vi "Update Lua Palettes.vi"() -> ()   [LabVIEW 2020, in "Lua DevUtil.lvlib"]
uses:
  Lua DevUtil.lvlib
  <vilib>/Utility/miscctls.llb/LVMapReplaceAction.ctl
  <vilib>/Palette API/Palette Menu/Public Type Define/Palette Data.ctl
  <vilib>/Palette API/Palette Menu/Public Type Define/View Format.ctl
  <vilib>/Palette API/Palette Menu/Public Type Define/Items.ctl
  <vilib>/Palette API/Palette Menu/Public Type Define/Item.ctl
  <vilib>/Palette API/Palette Menu/Public Type Define/Help Info.ctl
  <vilib>/Palette API/Palette Menu/Public Type Define/Synchronize Info.ctl
  <vilib>/Palette API/Palette Menu/Public Type Define/Palette type.ctl
  85e9b90b-9151-4f09-9030-f452b0e3cf19.vi
  <vilib>/Comparison/Less/Less Functor/Less Functor.lvclass
  <vilib>/Palette API/Palette Menu/Palette Menu.lvlib
panel:
  out "errors":T1(array[cluster])
  out "Lua menus":T2(c390)
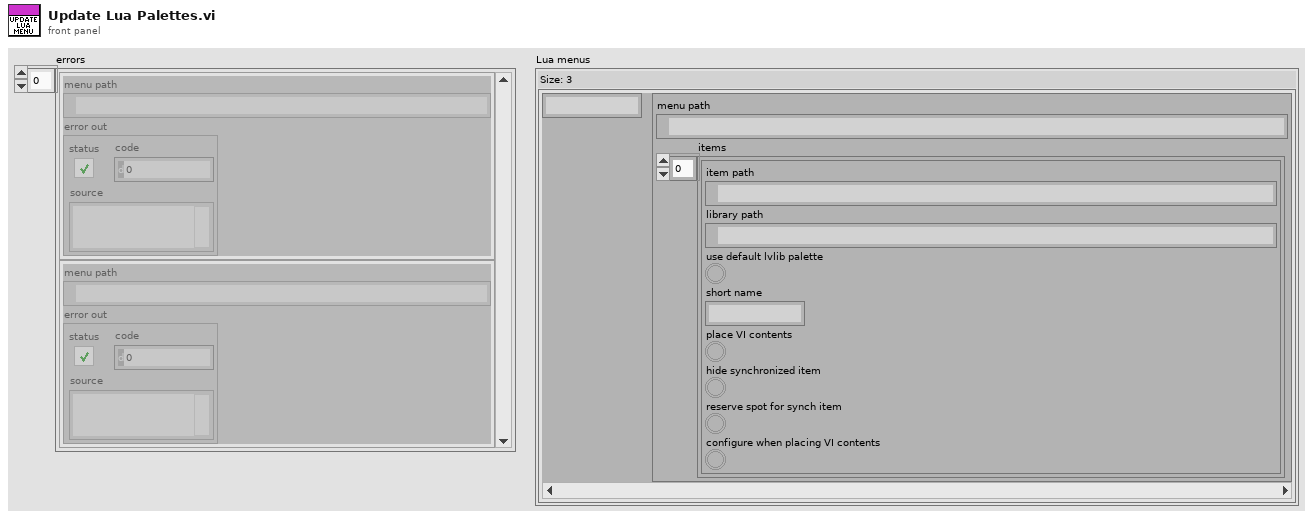
[diagram p1: front panel]
types:
  T1 = cluster{"menu path":path, "error out":errorcluster}[]
  T2 = map{string, cluster{"menu path":path, "items":cluster{"item path":path, "library path":path, "use default lvlib palette":bool, "short name":string, "place VI contents":bool, "hide synchronized item":bool, "reserve spot for synch item":bool, "configure when placing VI contents":bool}[]}}
  T3 = cluster{"item path":path, "library path":path, "use default lvlib palette":bool, "short name":string, "place VI contents":bool, "hide synchronized item":bool, "reserve spot for synch item":bool, "configure when placing VI contents":bool}
  T4 = typedef "LVMapReplaceAction.ctl" = enum32{"Modify Entry only if found", "Add or Modify Entry", "Delete Entry"}
  T5 = cluster{"menu path":path, "items":cluster{"item path":path, "library path":path, "use default lvlib palette":bool, "short name":string, "place VI contents":bool, "hide synchronized item":bool, "reserve spot for synch item":bool, "configure when placing VI contents":bool}[]}
  T6 = cluster{"item path":path, "library path":path, "use default lvlib palette":bool, "short name":string, "place VI contents":bool, "hide synchronized item":bool, "reserve spot for synch item":bool, "configure when placing VI contents":bool}[]
  T7 = typedef "Palette Menu.lvlib/View Format.ctl" = u16
  T8 = typedef "Palette Menu.lvlib/Palette Data.ctl" = cluster{"display name":string, "view format":T7, "palette width":i16, "items":T9, "256 color icon":picture, "B&W color icon":picture, "help information":T11, "palette description":string, "synchronize information":T12}
  T9 = typedef "Palette Menu.lvlib/Items.ctl" = T10[]
  T10 = typedef "Palette Menu.lvlib/Item.ctl" = cluster{"item path":path, "library path":path, "use default lvlib palette":bool, "short name":string, "place VI contents":bool, "hide synchronized item":bool, "reserve spot for synch item":bool, "configure when placing VI contents":bool}
  T11 = typedef "Palette Menu.lvlib/Help Info.ctl" = cluster{"help tag":string, "help file path ":path}
  T12 = typedef "Palette Menu.lvlib/Synchronize Info.ctl" = cluster{"synchronize with directory":bool, "synchronize directory path":path}
  T13 = typedef "Palette Menu.lvlib/Palette type.ctl" = i32
  T14 = cluster{"menu path":path, "error out":errorcluster}
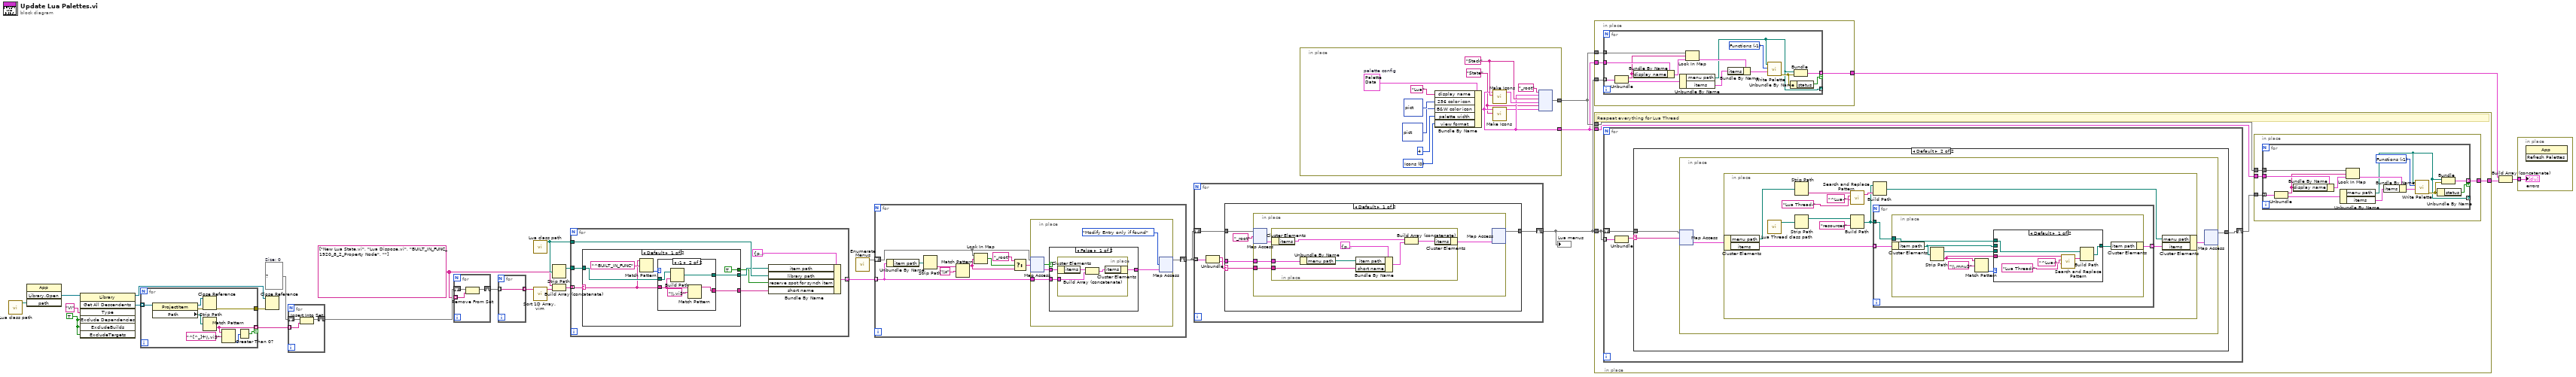
[diagram p0: block diagram]
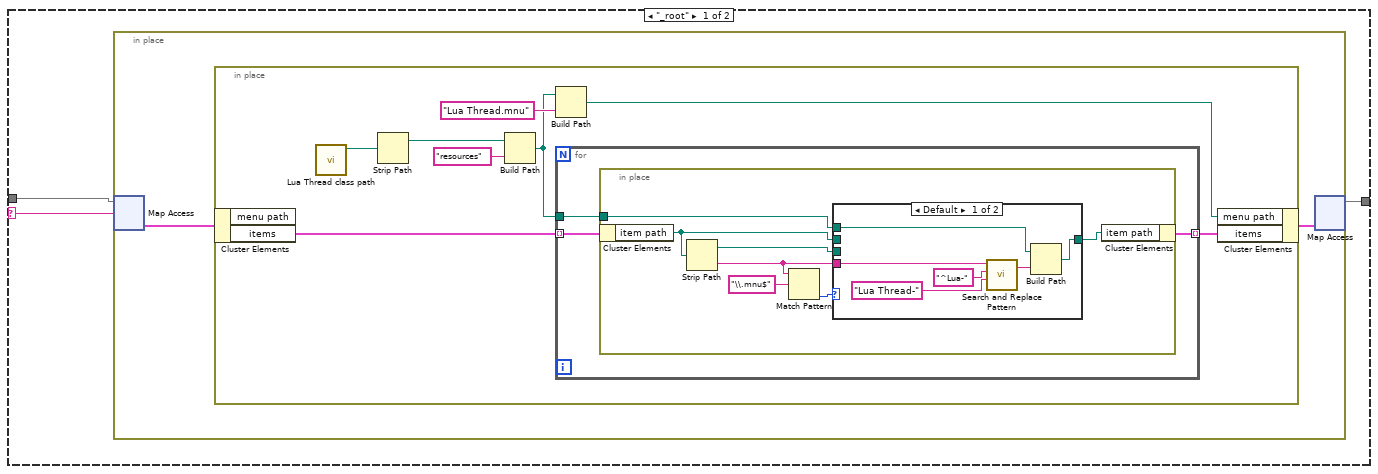
[diagram p2: hidden frame]
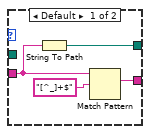
[diagram p7: hidden frame]
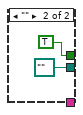
[diagram p8: hidden frame]
diagram:
  w17 = set{string} {}  # Size: 0
  w22 = TRUE ("ExcludeDependencies")
  w7 = string[] ["New Lua State.vi", "Lua Dispose.vi", "BUILT_IN_FUNC_1920_8_2_Property Node", ""]
  n1 = call "Lua class path.vi"() -> ("palette file path"=w25:path)  [unwired: 11 in]
  n2 = invoke class="App" method="Library.Open"("path"=w25) -> ("Open Library"=w24:refnum<vi>)  [unwired: 3 in, 3 out]
  n3 = invoke class="Library" method="Get All Descendents"(reference=w24, "Type"="VI", "Exclude Dependencies"=w22, "ExcludeBuilds"=w22, "ExcludeTargets"=w22) -> (reference out=w20:refnum<vi>, "All Descendents"=w21:refnum<vi>[])  [unwired: 2 in, 5 out]
  n4 = for {
    tunnel: w21 -> [w35] mode=indexing
    tunnel: [w27] -> w18 mode=indexing if=w29
    tunnel: [w32] -> w19
    n5 = property class="ProjectItem"(reference=w35) -> (reference out=w33:refnum<vi>, error out=w34:errorcluster, "Path"=w28:path)  [unwired: 1 in]
    n6 = Close Reference(reference=w33, error in (no error)=w34) -> (error out=w32:errorcluster)
    n7 = Strip Path(path=w28) -> (name=w27:string)  [unwired: 1 out]
    n8 = Match Pattern(string=w27, regular expression="^[^_]+\\.vi$") -> (offset past match=w30:i32)  [unwired: 1 in, 3 out]
    n9 = Greater Than 0?(x=w30) -> (x > 0?=w29:bool)
  }
  n10 = Close Reference(reference=w20, error in (no error)=w19) -> ()  [unwired: 1 out]
  n11 = for {
    shift-right: [w38] -> w16
    shift-left: w17 -> [w36]
    tunnel: w18 -> [w37] mode=indexing
    n12 = Insert Into Set(10:w37, 11:w36) -> (3:w38:set{string})  [unwired: 1 out]
  }
  n13 = for {
    shift-right: [w40] -> w15
    shift-left: w16 -> [w41]
    tunnel: w7 -> [w39] mode=indexing
    n14 = Remove From Set(10:w39, 11:w41) -> (3:w40:set{string})  [unwired: 1 out]
  }
  n15 = for {
    tunnel: w15 -> [w42] mode=indexing
    tunnel: [w42] -> w14 mode=indexing
  }
  n16 = call "Lua class path.vi"() -> ("palette file path"=w26:path)  [unwired: 11 in]
  n17 = call "Sort 1D Array.vim"("unsorted array"=w14) -> ("sorted array"=w13:string[])  [unwired: 10 in]
  n18 = Strip Path(path=w26) -> (stripped path=w11:path)  [unwired: 1 out]
  n19 = Build Array (concatenate)(w7, w13) -> (w12:string[])
  n20 = for {
    tunnel: w12 -> [w48] mode=indexing
    tunnel: [w49] -> w9 mode=indexing
    tunnel: w26 -> [w47]
    tunnel: w11 -> [w46]
    n21 = case shown="Default" w48 {
      selector: w48 -> [w54 _]
      tunnel: w46 -> [w57 _]
      tunnel: [w53 path "" ("appended path")] -> w45
      tunnel: [w52 _] -> w44
      tunnel: [TRUE ("use default lvlib palette") TRUE ("use default lvlib palette")] -> w43
      frame Default {
        n22 = Match Pattern(string=w54, regular expression="^BUILT_IN_FUNC") -> (offset past match=w55:i32)  [unwired: 1 in, 3 out]
        n23 = case shown="-1" w55 {
          tunnel: w57 -> [_ w66]
          tunnel: w54 -> [w60 w64]
          tunnel: [w61 w65] -> w53
          tunnel: [w58 w62] -> w52
          frame Default {
            n24 = String To Path(string=w60) -> (path=w61:path)
            n25 = Match Pattern(string=w60, regular expression="[^_]+$") -> (match substring=w58:string)  [unwired: 1 in, 3 out]
          }
          frame -1 {
            n26 = Build Path(base path=w66, name or relative path=w64) -> (appended path=w65:path)
            n27 = Match Pattern(string=w64, regular expression="\\.vi$") -> (before substring=w62:string)  [unwired: 1 in, 3 out]
          }
        }
      }
      frame "" {
      }
    }
    n28 = Bundle By Name(cluster=T3 {"item path"=path "", "library path"=path "", "use default lvlib palette"=FALSE, "short name"="", "place VI contents"=FALSE, "hide synchronized item"=FALSE, "reserve spot for synch item"=TRUE, "configure when placing VI contents"=FALSE}, "item path"=w45, "library path"=w47, "reserve spot for synch item"=w43, "short name"=w44) -> (w49:T3)
  }
  n29 = call "Enumerate Menus.vi"() -> ("Lua menus"=w10:T2)  [unwired: 11 in]
  n30 = for {
    shift-right: [w75] -> w8
    shift-left: w10 -> [w73]
    tunnel: w9 -> [w74] mode=indexing
    n31 = Unbundle By Name(w74) -> ("item path"=w78:path)
    n32 = Strip Path(path=w78) -> (name=w77:string)  [unwired: 1 out]
    n33 = Match Pattern(string=w77, regular expression="\\s") -> (before substring=w71:string)  [unwired: 1 in, 3 out]
    n34 = Look In Map(map=w73, key=w71) -> (key not found?=w72:bool)  [unwired: 1 in, 1 out]
    n35 = Select(t="_root" ("regular expression"), s=w72, f=w71) -> (s? t:f=w69:string)
    n36 = in-place {
      in-place-border: w74 -> [w79]
      n37 = in-place-map #1(w73, w69) -> (w81:T5, w83:bool)  [unwired: 1 in]
      n38 = case shown="False" w83 {
        tunnel: [w84 w90] -> w82
        tunnel: w81 -> [w86 w90]
        tunnel: w79 -> [w85 _]
        frame False {
          n39 = in-place {
            in-place-border: w85 -> [w88]
            n40 = in-place-cluster #2(w86) -> ("items"=w89:T6)
            n41 = Build Array (concatenate)(w89, w88) -> (w87:T6)
            n42 = in-place-cluster #2("items"=w87) -> (w84:T5)
          }
        }
        frame True {
        }
      }
      n43 = in-place-map #1(w82, LVMapReplaceAction."Modify Entry only if found" ("action")) -> (w75:T2)  [unwired: 2 out]
    }
  }
  n44 = for {
    tunnel: w8 -> [w95] mode=indexing
    shift-right: [w92] -> w5
    shift-left: w8 -> [w93]
    n45 = Unbundle(w95) -> ("submatch 1"=w94:string, w91:T5)
    n46 = case shown="Default" w94 {
      selector: w94 -> [w97 _]
      tunnel: w93 -> [w100 w112]
      tunnel: [w98 w112] -> w92
      tunnel: w91 -> [w99 _]
      frame Default {
        n47 = in-place {
          in-place-border: w99 -> [w103]
          in-place-border: w97 -> [w101]
          n48 = in-place-map #3(w100, "_root") -> (w104:T5)  [unwired: 1 in, 1 out]
          n49 = in-place {
            in-place-border: w103 -> [w111]
            in-place-border: w101 -> [w106]
            n50 = in-place-cluster #4(w104) -> ("items"=w110:T6)
            n51 = Unbundle By Name(w111) -> ("menu path"=w107:path)
            n52 = Bundle By Name(cluster=T3 {"item path"=path "", "library path"=path "", "use default lvlib palette"=FALSE, "short name"="", "place VI contents"=FALSE, "hide synchronized item"=FALSE, "reserve spot for synch item"=FALSE, "configure when placing VI contents"=FALSE}, "item path"=w107, "short name"=w106) -> (w105:T3)
            n53 = Build Array (concatenate)(w110, w105) -> (w109:T6)
            n54 = in-place-cluster #4("items"=w109) -> (w102:T5)
          }
          n55 = in-place-map #3(w102) -> (w98:T2)  [unwired: 1 in, 2 out]
        }
      }
      frame "_root" {
      }
    }
  }
  "Lua menus" <- w5
  n56 = in-place {
    in-place-border: [w119] -> w2
    in-place-border: [w115] -> w1
    w114 = "State" ("key")
    w118 = T7 0 items=["Icons", "Text", "Icons and Text"] ("view format")
    w116 = "Stack" ("key")
    w125 = T8 {"display name"="Lua", "view format"=0, "palette width"=2, "items"=[], "256 color icon"=bytes[1182], "B&W color icon"=bytes[286], "help information"={"help tag"="", "help file path "=path ""}, "palette description"="", "synchronize information"={"synchronize with directory"=FALSE, "synchronize directory path"=path ""}}  # palette config
    n57 = Bundle By Name(cluster=w125, "display name"="Lua", "256 color icon"=picture bytes[1182], "B&W color icon"=picture bytes[286], "palette width"=i16 4, "view format"=w118) -> (w115:T8)
    n58 = call "Make Icons.vi"("Display Name"=w116, "palette config in"=w115) -> ("palette config out"=w117:T8)  [unwired: 9 in]
    n59 = call "Make Icons.vi"("Display Name"=w114, "palette config in"=w115) -> ("palette config out"=w113:T8)  [unwired: 9 in]
    n60 = node("_root" ("key"), w115, w116, w117, w114, w113) -> (w119:map{string, T8})
  }
  n61 = in-place {
    in-place-border: [w129] -> w6
    in-place-border: w2 -> [w128]
    in-place-border: w1 -> [w127]
    in-place-border: w5 -> [w126]
    n62 = for {
      tunnel: w126 -> [w143] mode=indexing
      tunnel: w128 -> [w142]
      tunnel: w127 -> [w141]
      tunnel: [w134] -> w129 mode=indexing if=w133
      tunnel: [w130] -> _ mode=indexing
      w137 = T13 -1 items=["Functions"=-1, "Controls"=-2] ("palette type")
      n63 = Unbundle(w143) -> ("submatch 1"=w139:string, w138:T5)
      n64 = Bundle By Name(cluster=w141, "display name"=w139) -> (w140:T8)
      n65 = Unbundle By Name(w138) -> ("menu path"=w130:path, "items"=w135:T6)
      n66 = Look In Map(map=w142, key=w139, default value=w140) -> (value=w136:T8)  [unwired: 1 out]
      n67 = Bundle By Name(cluster=w136, "items"=w135) -> (w132:T8)
      n68 = call <vilib>:"Write Palette.vi"("palette data"=w132, "palette type"=w137, "palette path"=w130) -> ("error out"=w131:errorcluster)  [unwired: 8 in]
      n69 = Unbundle By Name(w131) -> ("status"=w133:bool)
      n70 = Bundle("menu path"=w130, "error out"=w131) -> (w134:T14)  [unwired: 1 in]
    }
  }
  n71 = in-place {
    in-place-border: w5 -> [w145]
    in-place-border: [w148] -> w3
    in-place-border: w2 -> [w147]
    in-place-border: w1 -> [w146]
    # "Reapeat everything for Lua Thread"
    n72 = for {
      tunnel: w145 -> [w152] mode=indexing
      shift-right: [w149] -> w144
      shift-left: w145 -> [w150]
      n73 = Unbundle(w152) -> ("submatch 1"=w151:string)  [unwired: 1 out]
      n74 = case shown="Default" w151 {
        selector: w151 -> [w154 w184]
        tunnel: w150 -> [w155 w185]
        tunnel: [w153 w183] -> w149
        frame "_root" {
          n75 = in-place {
            n76 = in-place-map #5(w155, w154) -> (w157:T5)  [unwired: 1 in, 1 out]
            n77 = in-place {
              n78 = in-place-cluster #6(w157) -> ("items"=w165:T6)  [unwired: 1 out]
              n79 = call "Lua Thread class path.vi"() -> ("Lua Thread Class Path"=w162:path)  [unwired: 11 in]
              n80 = Strip Path(path=w162) -> (stripped path=w163:path)  [unwired: 1 out]
              n81 = Build Path(base path=w163, name or relative path="resources" ("name")) -> (appended path=w158:path)
              n82 = Build Path(base path=w158, name or relative path="Lua Thread.mnu" ("regular expression (\"\")")) -> (appended path=w159:path)
              n83 = for {
                tunnel: w165 -> [w168] mode=indexing
                tunnel: [w167] -> w164 mode=indexing
                tunnel: w158 -> [w166]
                n84 = in-place {
                  in-place-border: w166 -> [w169]
                  n85 = in-place-cluster #7(w168) -> ("item path"=w172:path)
                  n86 = Strip Path(path=w172) -> (stripped path=w171:path, name=w170:string)
                  n87 = Match Pattern(string=w170, regular expression="\\.mnu$") -> (offset past match=w174:i32)  [unwired: 1 in, 3 out]
                  n88 = case shown="Default" w174 {
                    tunnel: [w177 w182] -> w173
                    tunnel: w172 -> [_ w182]
                    tunnel: w171 -> [_ _]
                    tunnel: w170 -> [w179 _]
                    tunnel: w169 -> [w176 _]
                    frame Default {
                      n89 = call <vilib>:"Search and Replace Pattern.vi"("string"=w179, "regular expression (\"\")"="^Lua-" ("regular expression (\"\")"), "replace string (\"\")"="Lua Thread-" ("regular expression (\"\")")) -> ("result string"=w178:string)  [unwired: 2 in, 1 out]
                      n90 = Build Path(base path=w176, name or relative path=w178) -> (appended path=w177:path)
                    }
                    frame -1 {
                    }
                  }
                  n91 = in-place-cluster #7("item path"=w173) -> (w167:T3)
                }
              }
              n92 = in-place-cluster #6("menu path"=w159, "items"=w164) -> (w156:T5)
            }
            n93 = in-place-map #5(w156) -> (w153:T2)  [unwired: 1 in, 2 out]
          }
        }
        frame Default {
          n94 = in-place {
            n95 = in-place-map #8(w185, w184) -> (w187:T5)  [unwired: 1 in, 1 out]
            n96 = in-place {
              n97 = in-place-cluster #9(w187) -> ("menu path"=w191:path, "items"=w199:T6)
              n98 = call "Lua Thread class path.vi"() -> ("Lua Thread Class Path"=w196:path)  [unwired: 11 in]
              n99 = Strip Path(path=w191) -> (name=w190:string)  [unwired: 1 out]
              n100 = Strip Path(path=w196) -> (stripped path=w197:path)  [unwired: 1 out]
              n101 = call <vilib>:"Search and Replace Pattern.vi"("string"=w190, "regular expression (\"\")"="^Lua-" ("regular expression (\"\")"), "replace string (\"\")"="Lua Thread-" ("regular expression (\"\")")) -> ("result string"=w194:string)  [unwired: 2 in, 1 out]
              n102 = Build Path(base path=w197, name or relative path="resources" ("name")) -> (appended path=w189:path)
              n103 = Build Path(base path=w189, name or relative path=w194) -> (appended path=w188:path)
              n104 = for {
                tunnel: w199 -> [w202] mode=indexing
                tunnel: [w201] -> w198 mode=indexing
                tunnel: w189 -> [w200]
                n105 = in-place {
                  in-place-border: w200 -> [w203]
                  n106 = in-place-cluster #10(w202) -> ("item path"=w206:path)
                  n107 = Strip Path(path=w206) -> (stripped path=w205:path, name=w204:string)
                  n108 = Match Pattern(string=w204, regular expression="\\.mnu$") -> (offset past match=w208:i32)  [unwired: 1 in, 3 out]
                  n109 = case shown="Default" w208 {
                    tunnel: [w211 w216] -> w207
                    tunnel: w206 -> [_ w216]
                    tunnel: w205 -> [_ _]
                    tunnel: w204 -> [w213 _]
                    tunnel: w203 -> [w210 _]
                    frame Default {
                      n110 = call <vilib>:"Search and Replace Pattern.vi"("string"=w213, "regular expression (\"\")"="^Lua-" ("regular expression (\"\")"), "replace string (\"\")"="Lua Thread-" ("regular expression (\"\")")) -> ("result string"=w212:string)  [unwired: 2 in, 1 out]
                      n111 = Build Path(base path=w210, name or relative path=w212) -> (appended path=w211:path)
                    }
                    frame -1 {
                    }
                  }
                  n112 = in-place-cluster #10("item path"=w207) -> (w201:T3)
                }
              }
              n113 = in-place-cluster #9("menu path"=w188, "items"=w198) -> (w186:T5)
            }
            n114 = in-place-map #8(w186) -> (w183:T2)  [unwired: 1 in, 2 out]
          }
        }
      }
    }
    n115 = in-place {
      in-place-border: [w220] -> w148
      in-place-border: w147 -> [w219]
      in-place-border: w146 -> [w218]
      in-place-border: w144 -> [w217]
      n116 = for {
        tunnel: w217 -> [w234] mode=indexing
        tunnel: w219 -> [w233]
        tunnel: w218 -> [w232]
        tunnel: [w225] -> w220 mode=indexing if=w224
        tunnel: [w221] -> _ mode=indexing
        w228 = T13 -1 items=["Functions"=-1, "Controls"=-2] ("palette type")
        n117 = Unbundle(w234) -> ("submatch 1"=w230:string, w229:T5)
        n118 = Bundle By Name(cluster=w232, "display name"=w230) -> (w231:T8)
        n119 = Unbundle By Name(w229) -> ("menu path"=w221:path, "items"=w226:T6)
        n120 = Look In Map(map=w233, key=w230, default value=w231) -> (value=w227:T8)  [unwired: 1 out]
        n121 = Bundle By Name(cluster=w227, "items"=w226) -> (w223:T8)
        n122 = call <vilib>:"Write Palette.vi"("palette data"=w223, "palette type"=w228, "palette path"=w221) -> ("error out"=w222:errorcluster)  [unwired: 8 in]
        n123 = Unbundle By Name(w222) -> ("status"=w224:bool)
        n124 = Bundle("menu path"=w221, "error out"=w222) -> (w225:T14)  [unwired: 1 in]
      }
    }
  }
  n125 = Build Array (concatenate)(w6, w3) -> (w4:T1)
  n126 = in-place {
    in-place-border: w4 -> [w235]
    n127 = invoke class="App" method="Refresh Palettes"() -> ()  [unwired: 3 in, 3 out]
    "errors" <- w235
  }
